vi "Update Timestamp.vi"(8 "error in (no error)":errorcluster, 10 "XNET CAN Data in":T1[](array[typedef]) {"payload" format="%x"; "timestamp" format="%<%.7X\n%x>T"; "type" items=["CAN Data"=0, "CAN Remote"=1, "CAN Bus Error"=2, "CAN 2.0 Data"=8, "CAN FD Data"=16, "CAN FD+BRS Data"=24, "J1939 Data"=192, "Delay"=224, "Log Trigger"=225, "Start Trigger"=226]; "identifier" format="%x"}, 11 "XNET CAN RW in":refnum<class "XNET CAN RW.lvclass">) -> (0 "error out":errorcluster, 2 "XNET CAN Data out":T1[](array[typedef]) {"payload" format="%x"; "timestamp" format="%<%.7X\n%x>T"; "type" items=["CAN Data"=0, "CAN Remote"=1, "CAN Bus Error"=2, "CAN 2.0 Data"=8, "CAN FD Data"=16, "CAN FD+BRS Data"=24, "J1939 Data"=192, "Delay"=224, "Log Trigger"=225, "Start Trigger"=226]; "identifier" format="%x"})   [LabVIEW 2021, in "XNET CAN RW.lvclass"]
doc: "Update the timestamps from the CAN return so the represent the system time instead of the CAN HW time. This is helpful if trying to correlate the timestamps with operations on the system. The system time and the CAN time will drift unless additional hardware is used on the system to servo system time and the backplane together."
uses:
  XNET CAN RW.lvclass
  <vilib>/xnet/xnet.llb/XNET Frame CAN.ctl
  <vilib>/xnet/xnet.llb/XNET Frame Type CAN.ctl
  XNET CAN RW.lvclass/XNET CAN RW.ctl
  <vilib>/CIF Foundation/CIF Utilities/Time/System Time/LabVIEW Time to TAI Time.vi
  <vilib>/CIF Foundation/CIF Utilities/Time/System Time/Get System Time.vi
  <vilib>/xnet/xnet.llb/XNET Read.vi
  <vilib>/xnet/xnet.llb/XNET Read (State Time Current).vi
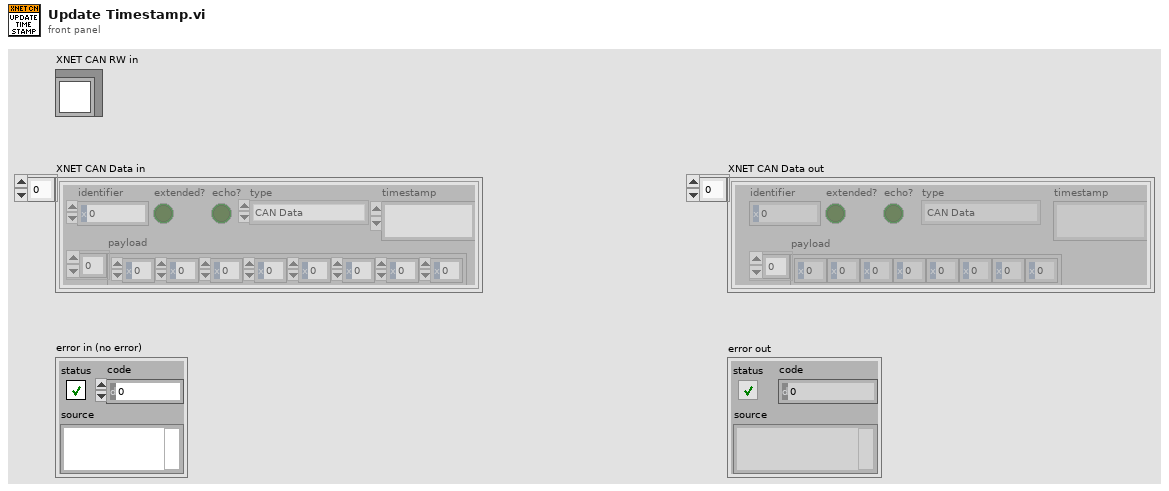
[diagram p1: front panel]
types:
  T1 = typedef "XNET Frame CAN.ctl" = cluster{"timestamp":timestamp, "payload":u8[], "identifier":u32, "type":T2, "extended?":bool, "echo?":bool}
  T2 = typedef "XNET Frame Type CAN.ctl" = u8
  T3 = typedef "XNET CAN RW.lvclass/Time Pair.ctl" = cluster{"System Time":i64, "CAN Time":i64}
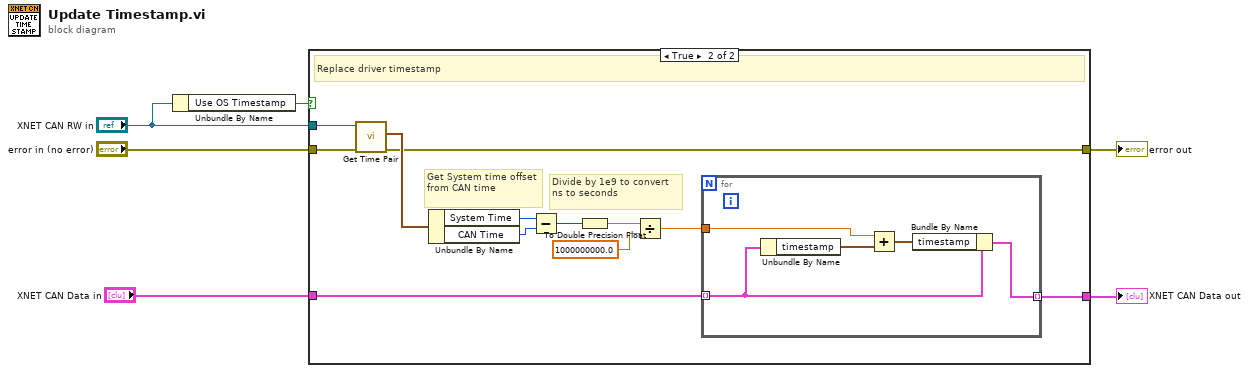
[diagram p0: block diagram]
diagram:
  n1 = Unbundle By Name("XNET CAN RW in") -> ("Use OS Timestamp"=w1:bool)
  n2 = case shown="True" w1 {
    tunnel: "XNET CAN Data in" -> [w8 w19]
    tunnel: [w8 w18] -> w5
    tunnel: "XNET CAN RW in" -> [_ w20]
    tunnel: "error in (no error)" -> [w7 w10]
    tunnel: [w7 w9] -> w3
    frame False {
      # "Don't replace driver timestamp"
    }
    frame True {
      # "Divide by 1e9 to convert ns to seconds"
      # "Get System time offset from CAN time"
      # "Replace driver timestamp"
      n3 = call "Get Time Pair.vi"("error in (no error)"=w10, "XNET CAN RW in"=w20) -> ("error out"=w9:errorcluster, "Time Pair"=w17:T3)  [unwired: 7 in, 1 out]
      n4 = Unbundle By Name(w17) -> ("System Time"=w16:i64, "CAN Time"=w15:i64)
      n5 = Subtract(x=w16, y=w15) -> (x-y=w14:i64)
      n6 = To Double Precision Float(number=w14) -> (double precision float=w11:dbl)
      n7 = Divide(x=w11, y=1000000000.0) -> (x/y=w12:dbl)
      n8 = for {
        tunnel: w19 -> [w24] mode=indexing
        tunnel: [w22] -> w18 mode=indexing
        tunnel: w12 -> [w21]
        n9 = Unbundle By Name(w24) -> ("timestamp"=w25:timestamp)
        n10 = Add(x=w21, y=w25) -> (x+y=w23:timestamp)
        n11 = Bundle By Name(cluster=w24, "timestamp"=w23) -> (w22:T1)
      }
    }
  }
  "XNET CAN Data out" <- w5
  "error out" <- w3
